vi "TEST_MenuRTM.vi"(10 "Color Theme":enum16{"LabVIEW", "Dark", "Windows Gray"}(ring), 11 "ExitEvent":refnum<user-event>) -> ()   [LabVIEW 2021, in "Menu.lvlib" / "Menu.lvclass"]
uses:
  Menu.lvclass
  Picture2D/src/Font/Font.lvclass
  Picture2D/src/Square/Square.lvclass
  C:/GitHub/Picture2D/src/Polygone/Polygone.lvclass
  C:/GitHub/Picture2D/src/Rectangle/Rectangle.lvclass
  C:/GitHub/Picture2D/src/Shape/Shape.lvclass
  C:/GitHub/Picture2D/src/Picture2D/Picture2D.lvclass
  Picture2D/src/Point/Point.lvclass
  Picture2D/src/Font/Font.lvclass/Font.ctl
  Picture2D/src/Color/Color.lvclass
  SubMenuIcon.ctl
  4d7882bf-4570-41b5-8159-e9b7f331f501.vi
  Picture2D/src/Font/SetFontName.vi
  Picture2D/src/Font/SetSize.vi
  SetBackgroundColor.vi
  SetBorderColor.vi
  SetHiliteColor.vi
  SetHiliteTextColor.vi
  SetTextColor.vi
  SetFont.vi
  SetDesiredFont.vi
  SetSubMenuIconType.vi
  SetSubMenuIconOpened.vi
  SetSubMenuIconClosed.vi
  <vilib>/ErrorRing/Error Ring.xnode
panel:
  out "2D Picture":picture
  in  "Font Name":string="Arial"
  in  "Size":i16=15
  in  "Desired Font":T1(ring)=enum."Application Font"
  out "ItemPath":string
  out "ItemTag":string
  out "error out":errorcluster
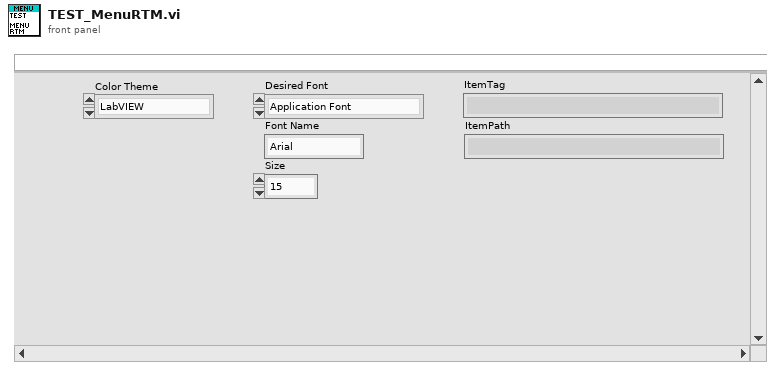
[diagram p1: front panel]
types:
  T1 = enum16{"User-specified Font", "Application Font", "System Font", "Dialog Font"}
  T2 = typedef "Menu.lvlib/Menu.lvclass/SubMenuIcon.ctl" = enum16{"LabVIEW", "Windows", "Custom"}
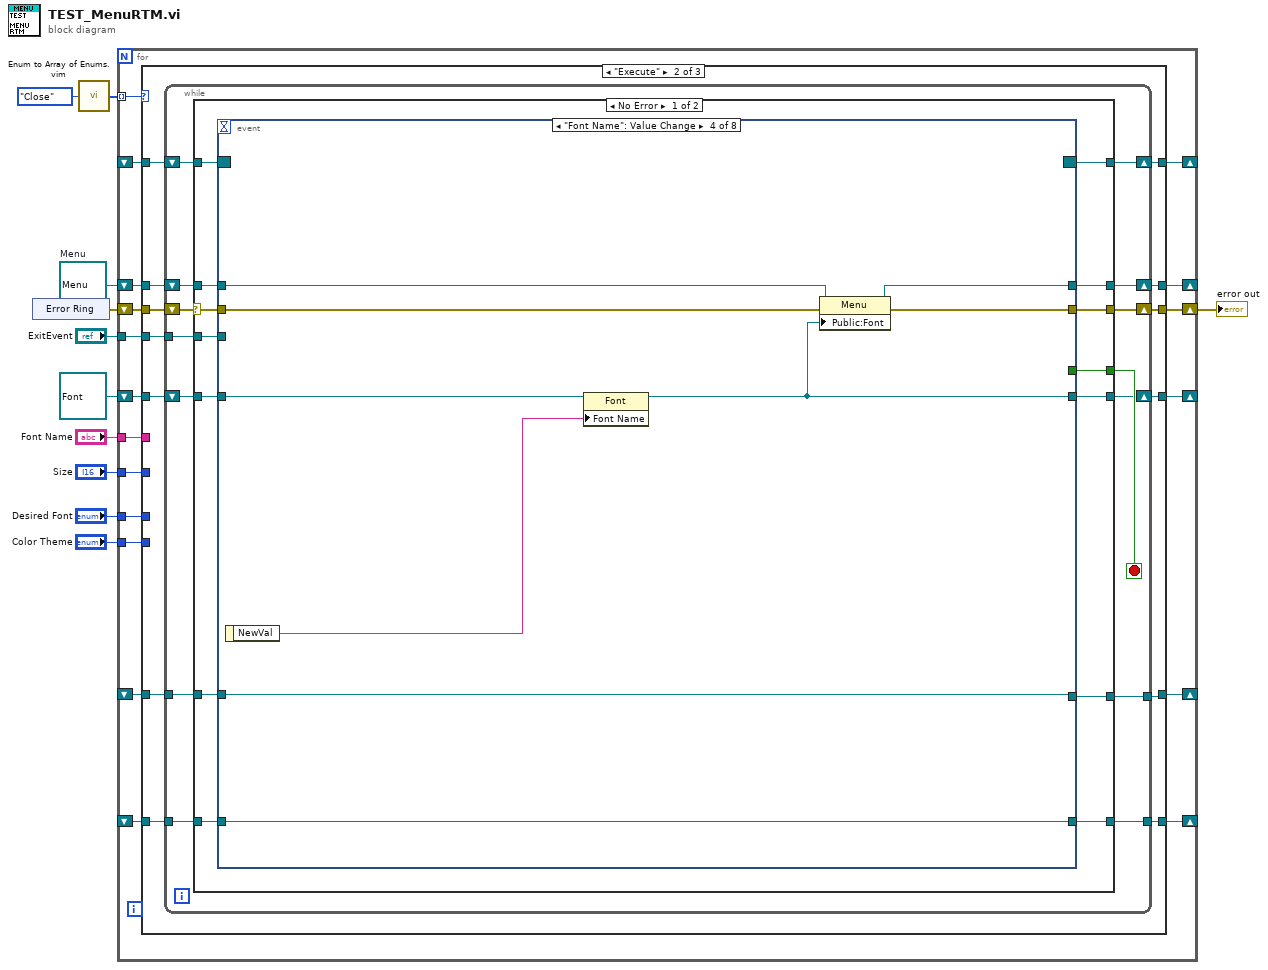
[diagram p0: block diagram]
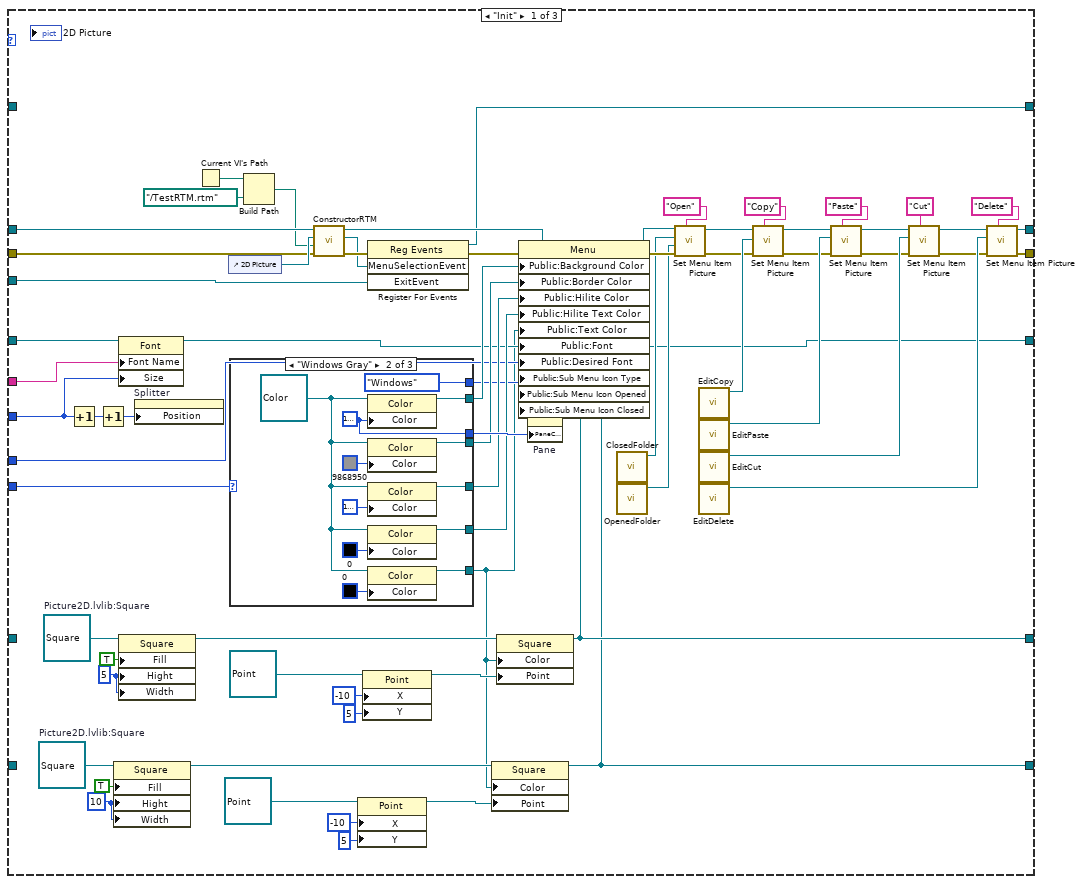
[diagram p2: hidden frame]
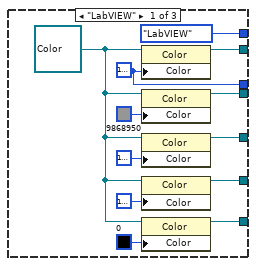
[diagram p3: hidden frame]
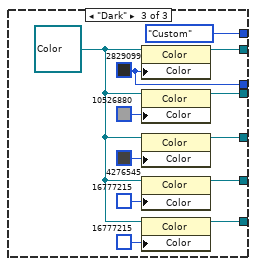
[diagram p4: hidden frame]
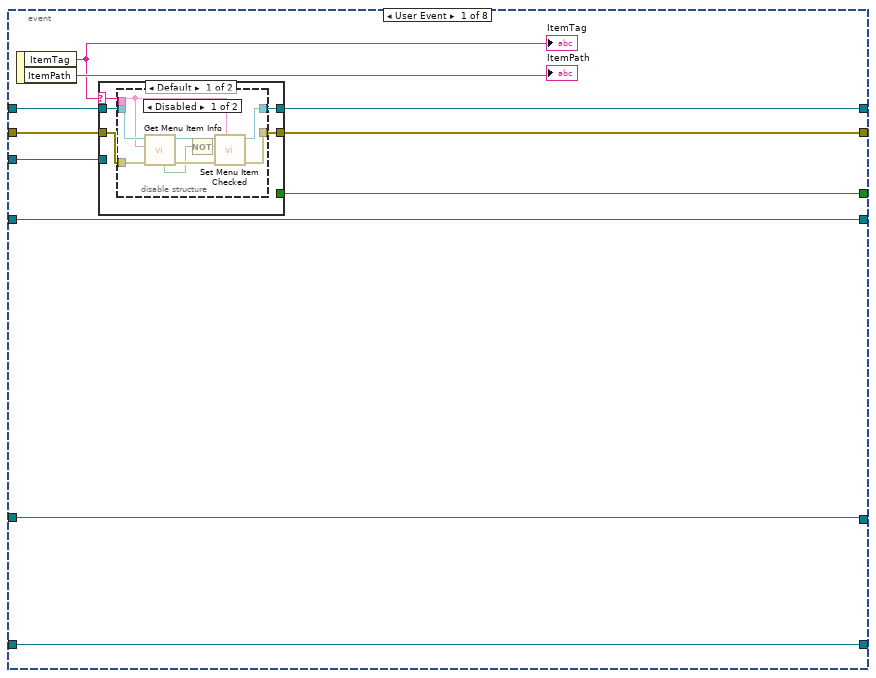
[diagram p5: hidden frame]
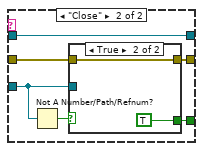
[diagram p7: hidden frame]
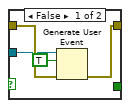
[diagram p8: hidden frame]
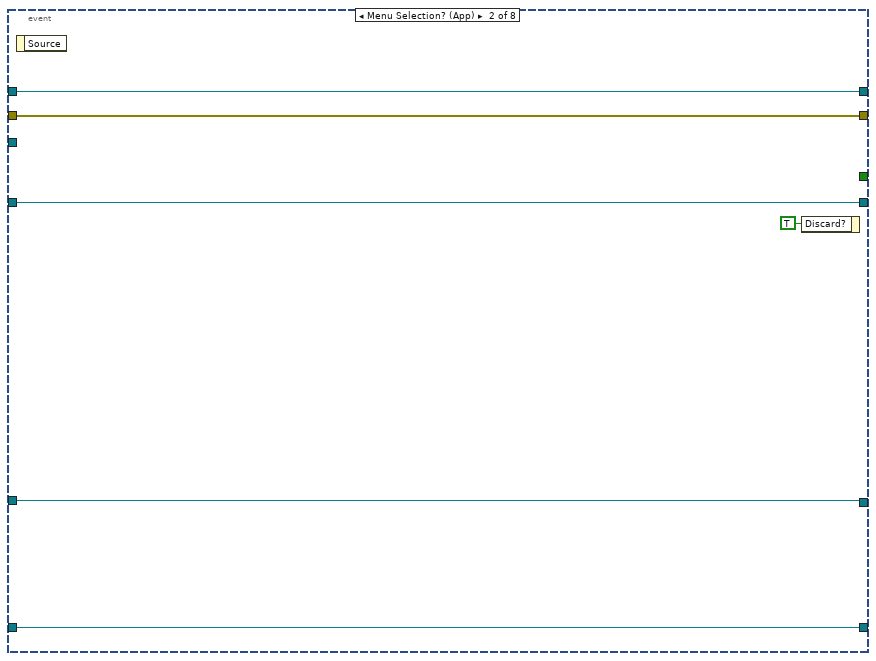
[diagram p9: hidden frame]
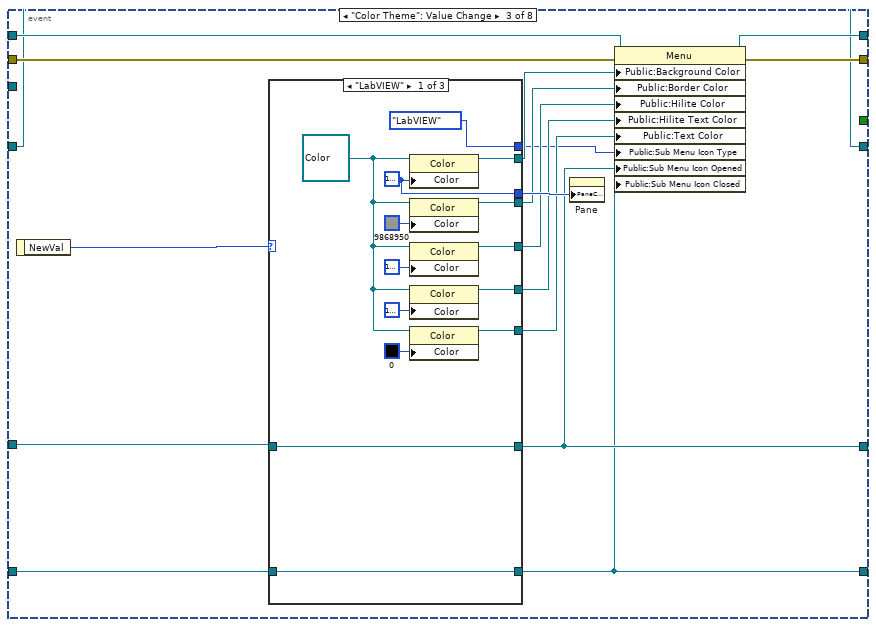
[diagram p10: hidden frame]
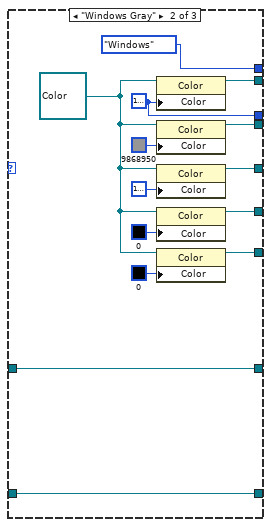
[diagram p11: hidden frame]
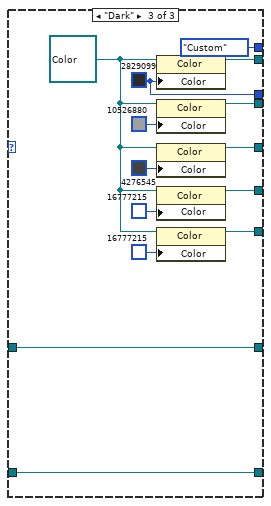
[diagram p12: hidden frame]
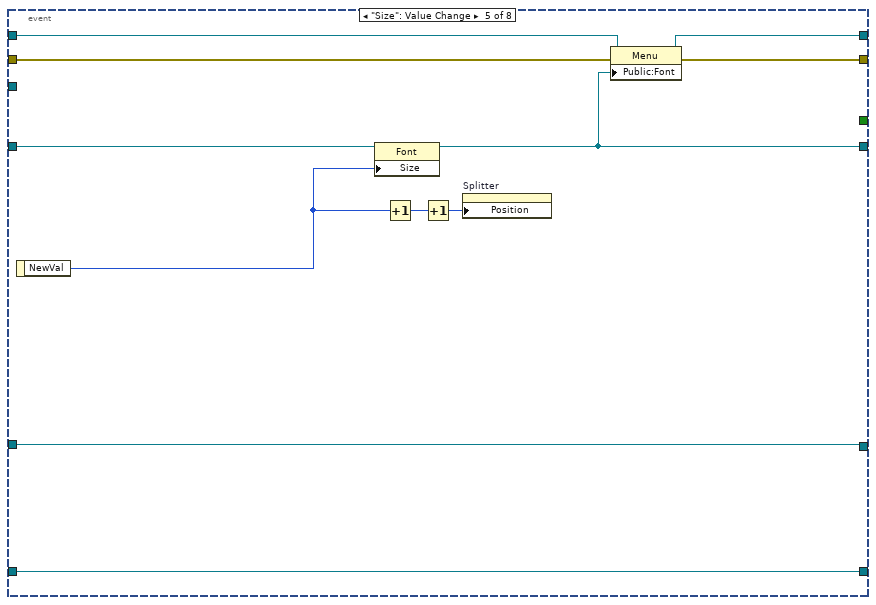
[diagram p13: hidden frame]
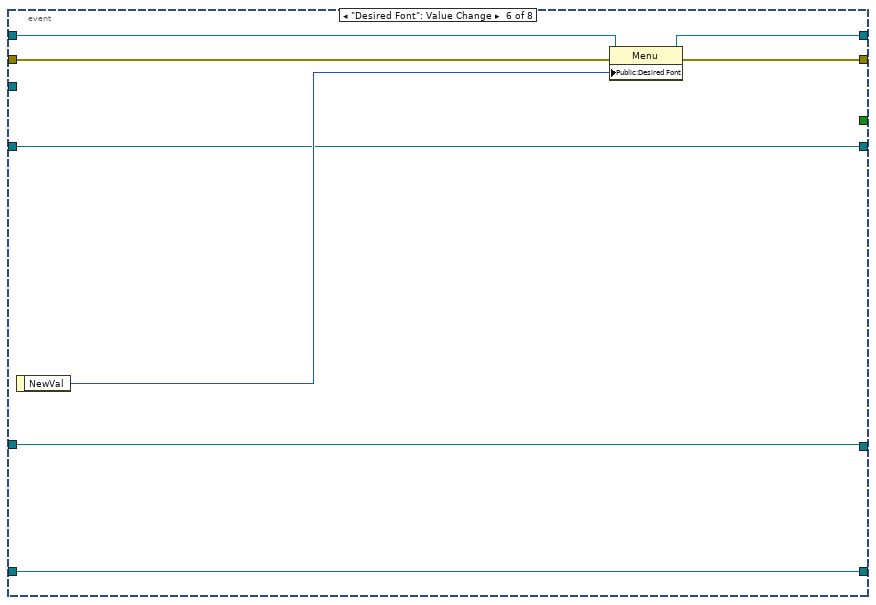
[diagram p14: hidden frame]
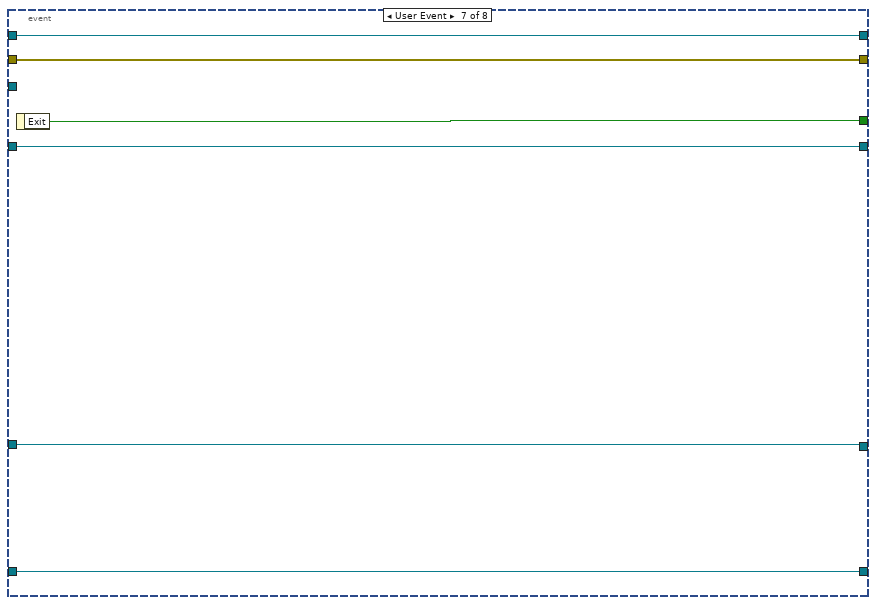
[diagram p15: hidden frame]
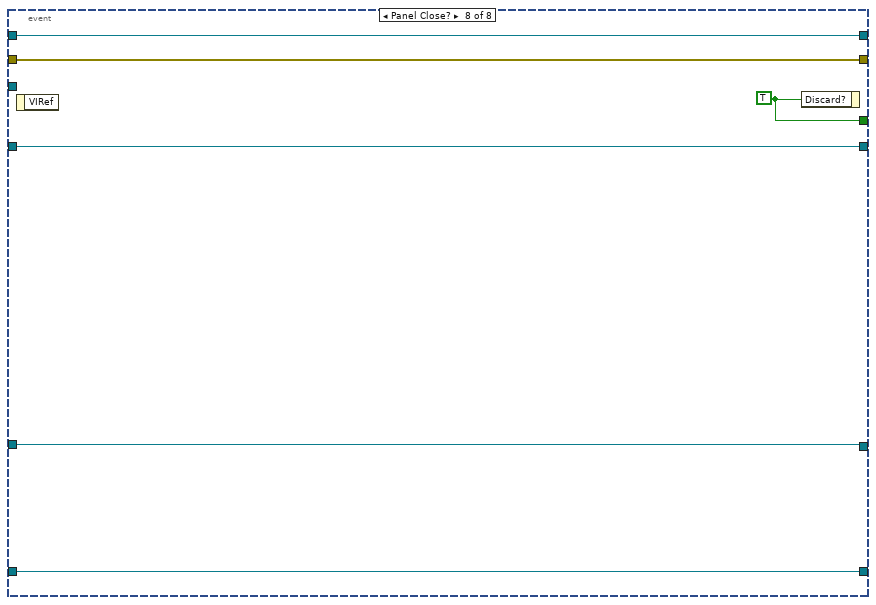
[diagram p16: hidden frame]
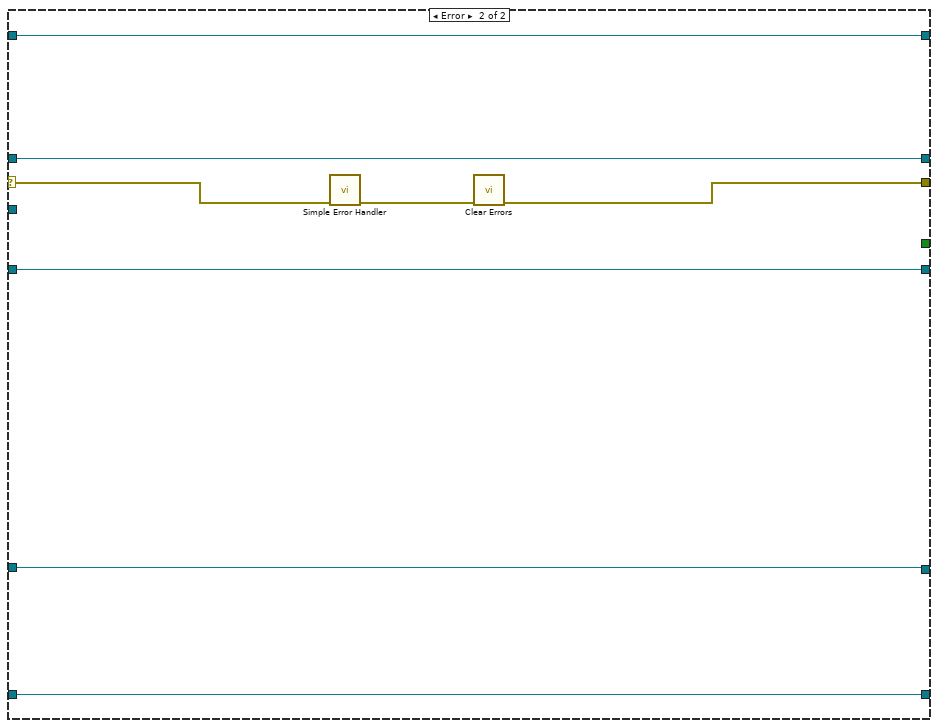
[diagram p17: hidden frame]
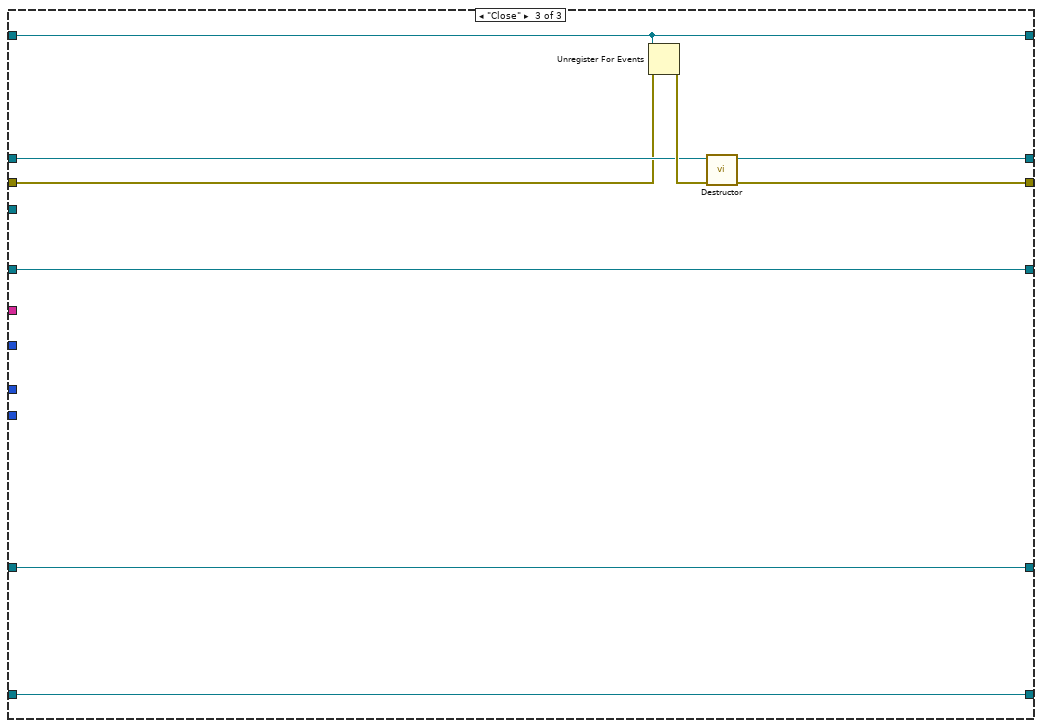
[diagram p18: hidden frame]
diagram:
  w3 = refnum<class "Menu.lvclass"> refnum  # Menu
  n1 = xnode "Error Ring"() -> ("error out"=w2:errorcluster)
  n2 = call "Enum to Array of Enums.vim"("enum"=enum16{"Init", "Execute", "Close"}."Close") -> ("array of enums"=w10:enum16{"Init", "Execute", "Close"}[])
  n3 = for {
    tunnel: "ExitEvent" -> [w26]
    shift-right: [w16] -> _
    shift-left: _ -> [w29]
    shift-right: [w18] -> w1
    shift-left: w2 -> [w28]
    shift-right: [w17] -> _
    shift-left: w3 -> [w27]
    tunnel: w10 -> [w25] mode=indexing
    tunnel: "Font Name" -> [w23]
    tunnel: "Size" -> [w22]
    tunnel: "Desired Font" -> [w21]
    tunnel: "Color Theme" -> [w20]
    shift-right: [w19] -> _
    shift-left: refnum<class "Font.lvclass"> refnum ("Fonts") -> [w24]
    shift-right: [w15] -> _
    shift-left: _ -> [w12]
    shift-right: [w14] -> _
    shift-left: _ -> [w13]
    n4 = case shown="\"Execute\"" w25 {
      tunnel: w29 -> [_ w146 w330]
      tunnel: [w61 w145 w331] -> w17
      tunnel: [w59 w144 w330] -> w16
      tunnel: [w60 w143 w333] -> w18
      tunnel: w28 -> [w53 w142 w329]
      tunnel: w27 -> [w62 w141 w331]
      tunnel: w26 -> [w58 w140 _]
      tunnel: w24 -> [w71 w139 w332]
      tunnel: w23 -> [w70 _ _]
      tunnel: w22 -> [w52 _ _]
      tunnel: w21 -> [w69 _ _]
      tunnel: w20 -> [w63 _ _]
      tunnel: [w57 w138 w332] -> w19
      tunnel: [w33 w135 w328] -> w15
      tunnel: [w32 w134 w327] -> w14
      tunnel: w13 -> [_ w136 w327]
      tunnel: w12 -> [_ w137 w328]
      frame "Init" {
        w37 = i16 10 ("Hight")
        w35 = refnum<class "Square.lvclass"> refnum  # Picture2D.lvlib:Square
        w48 = i16 5 ("Hight")
        w50 = refnum<class "Square.lvclass"> refnum  # Picture2D.lvlib:Square
        n5 = Increment(x=w52) -> (x+1=w31:i16)
        n6 = Increment(x=w31) -> (x+1=w30:i16)
        n7 = property class="Square"(reference=w35, "Fill"=TRUE, "Hight"=w37, "Width"=w37) -> (reference out=w42:refnum<class "Square.lvclass">)  [unwired: 1 in, 1 out]
        n8 = property class="Font"(reference=w71, "Font Name"=w70, "Size"=w52) -> (reference out=w57:refnum<class "Font.lvclass">)  [unwired: 1 in, 1 out]
        n9 = property class="Square"(reference=w50, "Fill"=TRUE, "Hight"=w48, "Width"=w48) -> (reference out=w43:refnum<class "Square.lvclass">)  [unwired: 1 in, 1 out]
        n10 = property on="Splitter" class="Splitter"("Position"=w30) -> ()  [unwired: 2 in, 2 out]
        n11 = Current VI's Path() -> (path=w56:path)
        n12 = control-ref of="2D Picture"() -> (w75:refnum<vi>)
        n13 = case shown="\"Windows Gray\"" w63 {
          tunnel: [w109 w121 w133] -> w77
          tunnel: [w107 w119 w131] -> w78
          tunnel: [w106 w118 w130] -> w79
          tunnel: [w105 w117 w129] -> w80
          tunnel: [w104 w116 w128] -> w34
          tunnel: [w99 w111 w123] -> w81
          tunnel: [SubMenuIcon."LabVIEW" ("SubMenuIconType") SubMenuIcon."Windows" ("SubMenuIconType") SubMenuIcon."Custom" ("SubMenuIconType")] -> w51
          frame "LabVIEW" {
            w99 = u32 16777238 ("Color")
            w108 = refnum<class "Color.lvclass"> refnum ("Background Color")
            n14 = property class="Color"(reference=w108, "Color"=w99) -> (reference out=w109:refnum<class "Color.lvclass">)  [unwired: 1 in, 1 out]
            n15 = property class="Color"(reference=w108, "Color"=u32 9868950) -> (reference out=w107:refnum<class "Color.lvclass">)  [unwired: 1 in, 1 out]
            n16 = property class="Color"(reference=w108, "Color"=u32 16777224) -> (reference out=w106:refnum<class "Color.lvclass">)  [unwired: 1 in, 1 out]
            n17 = property class="Color"(reference=w108, "Color"=u32 16777226) -> (reference out=w105:refnum<class "Color.lvclass">)  [unwired: 1 in, 1 out]
            n18 = property class="Color"(reference=w108, "Color"=u32 0) -> (reference out=w104:refnum<class "Color.lvclass">)  [unwired: 1 in, 1 out]
          }
          frame "Windows Gray" {
            w111 = u32 16777238 ("Color")
            w120 = refnum<class "Color.lvclass"> refnum ("Background Color")
            n19 = property class="Color"(reference=w120, "Color"=w111) -> (reference out=w121:refnum<class "Color.lvclass">)  [unwired: 1 in, 1 out]
            n20 = property class="Color"(reference=w120, "Color"=u32 9868950) -> (reference out=w119:refnum<class "Color.lvclass">)  [unwired: 1 in, 1 out]
            n21 = property class="Color"(reference=w120, "Color"=u32 16777225) -> (reference out=w118:refnum<class "Color.lvclass">)  [unwired: 1 in, 1 out]
            n22 = property class="Color"(reference=w120, "Color"=u32 0) -> (reference out=w117:refnum<class "Color.lvclass">)  [unwired: 1 in, 1 out]
            n23 = property class="Color"(reference=w120, "Color"=u32 0) -> (reference out=w116:refnum<class "Color.lvclass">)  [unwired: 1 in, 1 out]
          }
          frame "Dark" {
            w123 = u32 2829099 ("Color")
            w132 = refnum<class "Color.lvclass"> refnum ("Background Color")
            n24 = property class="Color"(reference=w132, "Color"=w123) -> (reference out=w133:refnum<class "Color.lvclass">)  [unwired: 1 in, 1 out]
            n25 = property class="Color"(reference=w132, "Color"=u32 10526880) -> (reference out=w131:refnum<class "Color.lvclass">)  [unwired: 1 in, 1 out]
            n26 = property class="Color"(reference=w132, "Color"=u32 4276545) -> (reference out=w130:refnum<class "Color.lvclass">)  [unwired: 1 in, 1 out]
            n27 = property class="Color"(reference=w132, "Color"=u32 16777215) -> (reference out=w129:refnum<class "Color.lvclass">)  [unwired: 1 in, 1 out]
            n28 = property class="Color"(reference=w132, "Color"=u32 16777215) -> (reference out=w128:refnum<class "Color.lvclass">)  [unwired: 1 in, 1 out]
          }
        }
        n29 = Build Path(base path=w56, name or relative path=path "../TestRTM.rtm") -> (appended path=w54:path)
        n30 = call "ConstructorRTM.vi"("error in (no error)"=w53, "RTM Path"=w54, "PictRef"=w75, "Menu in"=w62) -> ("error out"=w74:errorcluster, "MenuSelectionEvent"=w72:refnum<user-event>, "Menu out"=w76:refnum<class "Menu.lvclass">)  [unwired: 5 in]
        n31 = property class="Point"(reference=refnum<class "Point.lvclass"> refnum ("Point"), "X"=i16 -10, "Y"=i16 5) -> (reference out=w39:refnum<class "Point.lvclass">)  [unwired: 1 in, 1 out]
        n32 = property class="Point"(reference=refnum<class "Point.lvclass"> refnum ("Point"), "X"=i16 -10, "Y"=i16 5) -> (reference out=w46:refnum<class "Point.lvclass">)  [unwired: 1 in, 1 out]
        n33 = register-events(error in=w74, w72, w58) -> (reference out=w59:refnum<event-registration>, error out=w73:errorcluster)  [unwired: 1 in]
        n34 = property class="Square"(reference=w42, "Color"=w34, "Point"=w39) -> (reference out=w32:refnum<class "Square.lvclass">)  [unwired: 1 in, 1 out]
        n35 = property class="Square"(reference=w43, "Color"=w34, "Point"=w46) -> (reference out=w33:refnum<class "Square.lvclass">)  [unwired: 1 in, 1 out]
        n36 = property class="Menu"(reference=w76, error in=w73, "Public:Background Color"=w77, "Public:Border Color"=w78, "Public:Hilite Color"=w79, "Public:Hilite Text Color"=w80, "Public:Text Color"=w34, "Public:Font"=w57, "Public:Desired Font"=w69, "Public:Sub Menu Icon Type"=w51, "Public:Sub Menu Icon Opened"=w33, "Public:Sub Menu Icon Closed"=w32) -> (reference out=w96:refnum<class "Menu.lvclass">, error out=w97:errorcluster)
        n37 = property on="Pane" class="Pane"("PaneColor"=w81) -> ()  [unwired: 2 in, 2 out]
        n38 = call "ClosedFolder.vi"() -> ("Image out"=w94:refnum<class "Image.lvclass">)  [unwired: 11 in]
        n39 = call "OpenedFolder.vi"() -> ("Image out"=w95:refnum<class "Image.lvclass">)  [unwired: 11 in]
        n40 = call "Set Menu Item Picture.vi"("item tag"="Open", "error in (no error)"=w97, "Hilite Picture"=w95, "Picture"=w94, "Menu in"=w96) -> ("error out"=w83:errorcluster, "Menu out"=w82:refnum<class "Menu.lvclass">)  [unwired: 5 in]
        n41 = call "EditCopy.vi"() -> ("Image out"=w90:refnum<class "Image.lvclass">)  [unwired: 11 in]
        n42 = call "EditPaste.vi"() -> ("Image out"=w91:refnum<class "Image.lvclass">)  [unwired: 11 in]
        n43 = call "EditCut.vi"() -> ("Image out"=w92:refnum<class "Image.lvclass">)  [unwired: 11 in]
        n44 = call "EditDelete.vi"() -> ("Image out"=w93:refnum<class "Image.lvclass">)  [unwired: 11 in]
        n45 = call "Set Menu Item Picture.vi"("item tag"="Copy", "error in (no error)"=w83, "Picture"=w90, "Menu in"=w82) -> ("error out"=w85:errorcluster, "Menu out"=w84:refnum<class "Menu.lvclass">)  [unwired: 6 in]
        n46 = call "Set Menu Item Picture.vi"("item tag"="Paste", "error in (no error)"=w85, "Picture"=w91, "Menu in"=w84) -> ("error out"=w87:errorcluster, "Menu out"=w86:refnum<class "Menu.lvclass">)  [unwired: 6 in]
        n47 = call "Set Menu Item Picture.vi"("item tag"="Cut", "error in (no error)"=w87, "Picture"=w92, "Menu in"=w86) -> ("error out"=w89:errorcluster, "Menu out"=w88:refnum<class "Menu.lvclass">)  [unwired: 6 in]
        n48 = call "Set Menu Item Picture.vi"("item tag"="Delete", "error in (no error)"=w89, "Picture"=w93, "Menu in"=w88) -> ("error out"=w60:errorcluster, "Menu out"=w61:refnum<class "Menu.lvclass">)  [unwired: 6 in]
      }
      frame "Execute" {
        n49 = while {
          shift-right: [w158] -> w143
          shift-left: w142 -> [w159]
          shift-right: [w155] -> w144
          shift-left: w146 -> [w160]
          shift-right: [w156] -> w145
          shift-left: w141 -> [w157]
          tunnel: w140 -> [w153]
          shift-right: [w151] -> w138
          shift-left: w139 -> [w152]
          tunnel: w137 -> [w150]
          tunnel: w136 -> [w149]
          tunnel: [w148] -> w135
          tunnel: [w147] -> w134
          stop <- w154 stop-if-true
          n50 = case shown="No Error" w159 {
            selector: w159 -> [w173 w326]
            tunnel: w160 -> [w174 w325]
            tunnel: [w172 w322] -> w158
            tunnel: w157 -> [w171 w324]
            tunnel: [w170 w324] -> w156
            tunnel: [w169 w325] -> w155
            tunnel: [w168 _] -> w154
            tunnel: w153 -> [w167 _]
            tunnel: w152 -> [w166 w321]
            tunnel: [w165 w321] -> w151
            tunnel: w150 -> [w164 w320]
            tunnel: w149 -> [w163 w319]
            tunnel: [w162 w320] -> w148
            tunnel: [w161 w319] -> w147
            frame No Error {
              n51 = event shown="[3] \"Font Name\": Value Change" {
                selector: w174 -> [_ _ _ _ _ _ _ _]
                dyn-events: [_ _ _ _ _ _ _ _] -> w169
                timeout: _ -> [_ _ _ _ _ _ _ _]
                tunnel: [w182 w219 w229 w284 w296 w306 w312 w317] -> w172
                tunnel: w173 -> [w183 w219 w230 w283 w295 w305 w312 w317]
                tunnel: [w181 w218 w228 w282 w294 w304 w311 w316] -> w170
                tunnel: w171 -> [w184 w218 w227 w281 w293 w303 w311 w316]
                tunnel: [w179 _ _ _ _ _ w310 w318] -> w168
                tunnel: w167 -> [w180 _ _ _ _ _ _ _]
                tunnel: w166 -> [w178 w217 w225 w287 w298 w301 w309 w315]
                tunnel: [w178 w217 w225 w286 w297 w301 w309 w315] -> w165
                tunnel: w164 -> [w175 w214 w223 w279 w288 w300 w307 w313]
                tunnel: w163 -> [w176 w215 w222 w280 w289 w299 w308 w314]
                tunnel: [w175 w214 w221 w279 w288 w300 w307 w313] -> w162
                tunnel: [w176 w215 w220 w280 w289 w299 w308 w314] -> w161
                event User Event {
                  n52 = event-data() -> ("ItemTag"=w177:string, "ItemPath"=→"ItemPath":string)  [unwired: 1 in]
                  "ItemTag" <- w177
                  n53 = case shown="Default" w177 {
                    selector: w177 -> [w186 _]
                    tunnel: w184 -> [w190 w207]
                    tunnel: w183 -> [w189 w205]
                    tunnel: [w188 w206] -> w182
                    tunnel: [w187 w207] -> w181
                    tunnel: w180 -> [_ w204]
                    tunnel: [_ w202] -> w179
                    frame Default {
                      n54 = disable-structure shown="Disabled" {
                        disable-tunnel: w190 -> [w199 w200]
                        disable-tunnel: w189 -> [w198 w201]
                        disable-tunnel: [w196 w201] -> w188
                        disable-tunnel: [w194 w200] -> w187
                        disable-tunnel: w186 -> [w191 _]
                        frame Disabled {
                          n55 = call "Get Menu Item Info.vi"("error in (no error)"=w198, "item tag"=w191, "Menu in"=w199) -> ("error out"=w197:errorcluster, "Menu out"=w195:refnum<class "Menu.lvclass">, "checked"=w193:bool)  [unwired: 1 in, 5 out]
                          n56 = Not(x=w193) -> (.not. x?=w192:bool)
                          n57 = call "Set Menu Item Checked.vi"("item tag"=w191, "error in (no error)"=w197, "checked"=w192, "Menu in"=w195) -> ("error out"=w196:errorcluster, "Menu out"=w194:refnum<class "Menu.lvclass">)  [unwired: 6 in]
                        }
                        frame Enabled {
                        }
                      }
                    }
                    frame "Close" {
                      n58 = Not A Number/Path/Refnum?(number/path/refnum=w204) -> (NaN/Path/Refnum?=w203:bool)
                      n59 = case shown="True" w203 {
                        tunnel: [w211 w213] -> w206
                        tunnel: w205 -> [w210 w213]
                        tunnel: w204 -> [w208 _]
                        tunnel: [_ TRUE] -> w202
                        frame False {
                          n60 = Generate User Event(user event=w208, event data cluster=TRUE ("event data"), error in=w210) -> (error out=w211:errorcluster)  [unwired: 1 in, 1 out]
                        }
                        frame True {
                        }
                      }
                    }
                  }
                }
                event Menu Selection? (App) {
                  n61 = event-data() -> ()  [unwired: 1 in, 1 out]
                  n62 = event-data("Discard?"=TRUE) -> ()  [unwired: 1 in, 1 out]
                }
                event "Color Theme": Value Change {
                  n63 = event-data() -> ("NewVal"=w226:enum16{"LabVIEW", "Dark", "Windows Gray"})  [unwired: 1 in]
                  n64 = case shown="\"LabVIEW\"" w226 {
                    tunnel: [w250 w264 w278] -> w231
                    tunnel: [w248 w262 w276] -> w232
                    tunnel: [w247 w261 w275] -> w233
                    tunnel: [w246 w260 w274] -> w234
                    tunnel: [w245 w259 w273] -> w235
                    tunnel: [w240 w254 w268] -> w236
                    tunnel: [SubMenuIcon."LabVIEW" ("SubMenuIconType") SubMenuIcon."Windows" ("SubMenuIconType") SubMenuIcon."Custom" ("SubMenuIconType")] -> w224
                    tunnel: [w238 w252 w266] -> w221
                    tunnel: w223 -> [w238 w252 w266]
                    tunnel: [w237 w251 w265] -> w220
                    tunnel: w222 -> [w237 w251 w265]
                    frame "LabVIEW" {
                      w240 = u32 16777238 ("Color")
                      w249 = refnum<class "Color.lvclass"> refnum ("Background Color")
                      n65 = property class="Color"(reference=w249, "Color"=w240) -> (reference out=w250:refnum<class "Color.lvclass">)  [unwired: 1 in, 1 out]
                      n66 = property class="Color"(reference=w249, "Color"=u32 9868950) -> (reference out=w248:refnum<class "Color.lvclass">)  [unwired: 1 in, 1 out]
                      n67 = property class="Color"(reference=w249, "Color"=u32 16777224) -> (reference out=w247:refnum<class "Color.lvclass">)  [unwired: 1 in, 1 out]
                      n68 = property class="Color"(reference=w249, "Color"=u32 16777226) -> (reference out=w246:refnum<class "Color.lvclass">)  [unwired: 1 in, 1 out]
                      n69 = property class="Color"(reference=w249, "Color"=u32 0) -> (reference out=w245:refnum<class "Color.lvclass">)  [unwired: 1 in, 1 out]
                    }
                    frame "Windows Gray" {
                      w254 = u32 16777238 ("Color")
                      w263 = refnum<class "Color.lvclass"> refnum ("Background Color")
                      n70 = property class="Color"(reference=w263, "Color"=w254) -> (reference out=w264:refnum<class "Color.lvclass">)  [unwired: 1 in, 1 out]
                      n71 = property class="Color"(reference=w263, "Color"=u32 9868950) -> (reference out=w262:refnum<class "Color.lvclass">)  [unwired: 1 in, 1 out]
                      n72 = property class="Color"(reference=w263, "Color"=u32 16777225) -> (reference out=w261:refnum<class "Color.lvclass">)  [unwired: 1 in, 1 out]
                      n73 = property class="Color"(reference=w263, "Color"=u32 0) -> (reference out=w260:refnum<class "Color.lvclass">)  [unwired: 1 in, 1 out]
                      n74 = property class="Color"(reference=w263, "Color"=u32 0) -> (reference out=w259:refnum<class "Color.lvclass">)  [unwired: 1 in, 1 out]
                    }
                    frame "Dark" {
                      w268 = u32 2829099 ("Color")
                      w277 = refnum<class "Color.lvclass"> refnum ("Background Color")
                      n75 = property class="Color"(reference=w277, "Color"=w268) -> (reference out=w278:refnum<class "Color.lvclass">)  [unwired: 1 in, 1 out]
                      n76 = property class="Color"(reference=w277, "Color"=u32 10526880) -> (reference out=w276:refnum<class "Color.lvclass">)  [unwired: 1 in, 1 out]
                      n77 = property class="Color"(reference=w277, "Color"=u32 4276545) -> (reference out=w275:refnum<class "Color.lvclass">)  [unwired: 1 in, 1 out]
                      n78 = property class="Color"(reference=w277, "Color"=u32 16777215) -> (reference out=w274:refnum<class "Color.lvclass">)  [unwired: 1 in, 1 out]
                      n79 = property class="Color"(reference=w277, "Color"=u32 16777215) -> (reference out=w273:refnum<class "Color.lvclass">)  [unwired: 1 in, 1 out]
                    }
                  }
                  n80 = property on="Pane" class="Pane"("PaneColor"=w236) -> ()  [unwired: 2 in, 2 out]
                  n81 = property class="Menu"(reference=w227, error in=w230, "Public:Background Color"=w231, "Public:Border Color"=w232, "Public:Hilite Color"=w233, "Public:Hilite Text Color"=w234, "Public:Text Color"=w235, "Public:Sub Menu Icon Type"=w224, "Public:Sub Menu Icon Opened"=w221, "Public:Sub Menu Icon Closed"=w220) -> (reference out=w228:refnum<class "Menu.lvclass">, error out=w229:errorcluster)
                }
                event "Font Name": Value Change {
                  n82 = event-data() -> ("NewVal"=w285:string)  [unwired: 1 in]
                  n83 = property class="Font"(reference=w287, "Font Name"=w285) -> (reference out=w286:refnum<class "Font.lvclass">)  [unwired: 1 in, 1 out]
                  n84 = property class="Menu"(reference=w281, error in=w283, "Public:Font"=w286) -> (reference out=w282:refnum<class "Menu.lvclass">, error out=w284:errorcluster)
                }
                event "Size": Value Change {
                  n85 = event-data() -> ("NewVal"=w292:i16)  [unwired: 1 in]
                  n86 = property class="Font"(reference=w298, "Size"=w292) -> (reference out=w297:refnum<class "Font.lvclass">)  [unwired: 1 in, 1 out]
                  n87 = Increment(x=w292) -> (x+1=w291:i16)
                  n88 = Increment(x=w291) -> (x+1=w290:i16)
                  n89 = property on="Splitter" class="Splitter"("Position"=w290) -> ()  [unwired: 2 in, 2 out]
                  n90 = property class="Menu"(reference=w293, error in=w295, "Public:Font"=w297) -> (reference out=w294:refnum<class "Menu.lvclass">, error out=w296:errorcluster)
                }
                event "Desired Font": Value Change {
                  n91 = event-data() -> ("NewVal"=w302:T1)  [unwired: 1 in]
                  n92 = property class="Menu"(reference=w303, error in=w305, "Public:Desired Font"=w302) -> (reference out=w304:refnum<class "Menu.lvclass">, error out=w306:errorcluster)
                }
                event User Event {
                  n93 = event-data() -> ("Exit"=w310:bool)  [unwired: 1 in]
                }
                event Panel Close? {
                  w318 = TRUE ("Discard?")
                  n94 = event-data() -> ()  [unwired: 1 in, 1 out]
                  n95 = event-data("Discard?"=w318) -> ()  [unwired: 1 in, 1 out]
                }
              }
            }
            frame Error {
              n96 = call <vilib>:"Simple Error Handler.vi"("error in (no error)"=w326) -> ("error out"=w323:errorcluster)  [unwired: 4 in, 4 out]
              n97 = call <vilib>:"Clear Errors.vi"("error in (no error)"=w323) -> ("error out"=w322:errorcluster)  [unwired: 5 in, 1 out]
            }
          }
        }
      }
      frame "Close" {
        n98 = Unregister For Events(event registration refnum=w330, error in=w329) -> (error out=w334:errorcluster)
        n99 = call "Destructor.vi"("error in (no error)"=w334, "Menu in"=w331) -> ("error out"=w333:errorcluster)  [unwired: 9 in]
      }
    }
  }
  "error out" <- w1
